vi "ot-spectra-to-flexlogger-test.vi"(1 "Order Settings":T2={"pulses per rev"=1, "trigger level (V)"=2.5, "max order"=64.0, "order resolution"=0.1, "window"=1, "averaging parameters"={"averaging mode"=enum."No averaging", "weighting mode"=enum."Linear", "number of averages"=1, "linear mode"=enum."One shot"}, "order ranges"=[{"start"=0.8, "stop"=1.2}, {"start"=1.8, "stop"=2.2}, {"start"=3.37, "stop"=3.77}, {"start"=3.8, "stop"=4.2}, {"start"=23.8, "stop"=24.2}]}, 4 "Noise (g rms)":dbl=0.01, 5 "Phases (deg)":dbl[](array[numeric])=[30.0, 0.0, 0.0, 0.0, 0.0], 6 "Orders":dbl[](array[numeric])=[1.0, 2.0, 3.57, 4.0, 24.0], 7 "Amplitudes (g pk)":dbl[](array[numeric])=[0.5, 0.2, 0.1, 0.05, 0.3], 8 "error in (no error)":errorcluster, 9 "Duration (s)":dbl=30.0, 10 "Ramps":T3(array[cluster]), 11 "Base RPM":dbl=3000.0) -> (0 "error out":errorcluster, 2 "True RPM":dbl[](array[numeric]), 3 "Tach RPM":dbl[](array[numeric]))   [LabVIEW 2026]
doc: "Unit-test harness for OT Spectra to FlexLogger.vi, fed block by block by the S&V order power spectrum chain of the NI example (Analog Tacho Process, Convert to Even Angle, Order Power Spectrum). Synthesises accel (sum of order sines, peak amplitudes, uniform noise) and a 1 ppr 0-5 V square tach (rising edge at shaft angle 0) for rpm(t) = Base RPM + sum of linear ramps, cuts it into 0.1 s blocks (5120 S @ 51.2 kS/s) and calls OrderPowerSpectrum.vi block by block like FlexLogger Process.vi does (Data In = [accel, tach], reset? TRUE on block 0). Returns NUMERIC arrays only: Values [blocks x (2 + order ranges)] = RPM, order amplitudes (g rms), Spectrum Valid, True RPM at each block centre."
uses:
  <vilib>/addons/Sound and Vibration/Order Analysis/Tach Process/OAT Analog Tacho Process (1 Tacho).vi
  <vilib>/addons/Sound and Vibration/Order Analysis/Resample Order Tracking/OAT Convert to Even Angle Signal (1 Channel).vi
  <vilib>/addons/Sound and Vibration/Order Analysis/Resample Order Tracking/OAT Order Power Spectrum (1 Channel).vi
  <vilib>/addons/Sound and Vibration/Order Analysis/Tach Process/SoundVib_TachProcess.lvlib
  <vilib>/addons/Sound and Vibration/Order Analysis/Resample Order Tracking/SoundVib_OrderTracking.lvlib
panel:
  out "Waveforms per Block":i32[](array[numeric])
  out "Values":dbl[][](array[numeric])
  in  "Settings":T1={"channels"=1, "orders"=[1.0, 2.0, 24.0], "band half-width (orders)"=0.2, "window ENBW (bins)"=1.5}
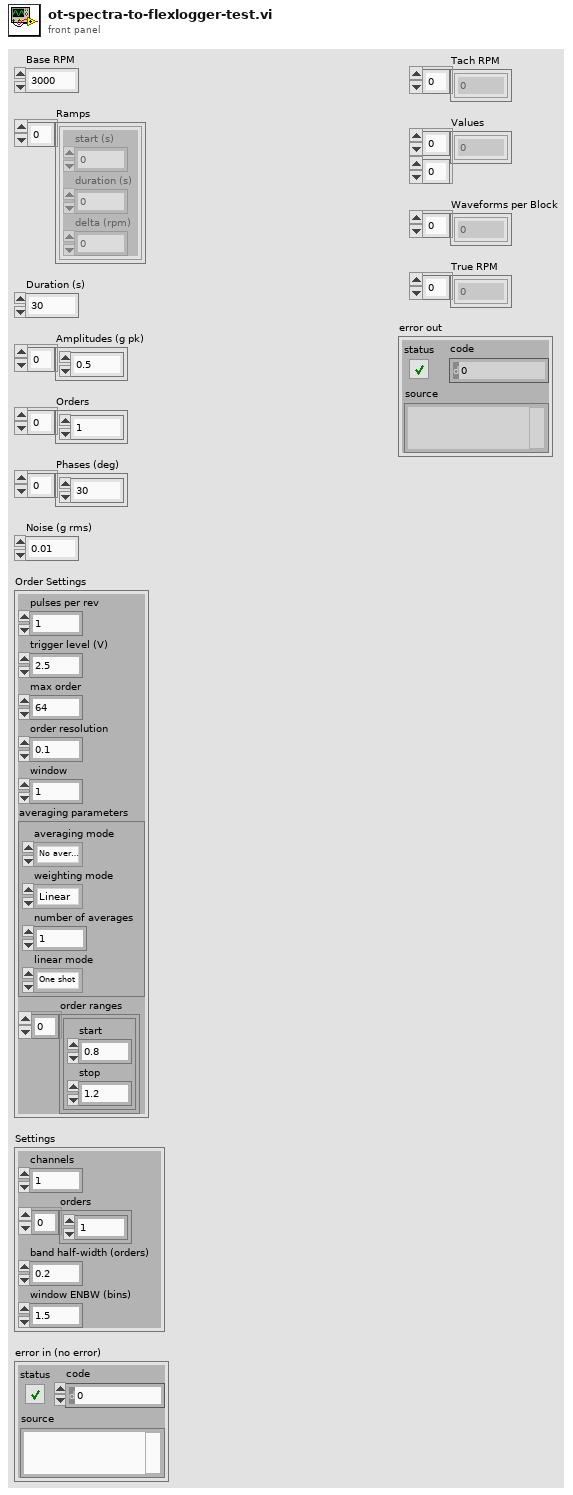
[diagram p1: front panel]
types:
  T1 = cluster{"channels":i32, "orders":dbl[], "band half-width (orders)":dbl, "window ENBW (bins)":dbl}
  T2 = cluster{"pulses per rev":i32, "trigger level (V)":dbl, "max order":dbl, "order resolution":dbl, "window":u32, "averaging parameters":cluster{"averaging mode":enum16{"No averaging", "Vector averaging", "RMS averaging", "Peak hold"}, "weighting mode":enum16{"Linear", "Exponential"}, "number of averages":u32, "linear mode":enum16{"One shot", "Auto restart"}}, "order ranges":cluster{"start":dbl, "stop":dbl}[]}
  T3 = cluster{"start (s)":dbl, "duration (s)":dbl, "delta (rpm)":dbl}[]
  T4 = cluster{"averaging mode":enum16{"No averaging", "Vector averaging", "RMS averaging", "Peak hold"}, "weighting mode":enum16{"Linear", "Exponential"}, "number of averages":u32, "linear mode":enum16{"One shot", "Auto restart"}}
  T5 = typedef "SoundVib_TachProcess.lvlib/speed profile.ctl" = cluster{"time [s]":dbl[], "speed [RPM]":dbl[]}
  T6 = typedef "svc_Resampled Channel Info.ctl" = cluster{"channel name":string, "description":string, " channel info":T7}
  T7 = typedef "svc_Channel Info.ctl" = cluster{"sensor sensitivity":dbl, "engineering units":T8, "dB reference":dbl, "custom label":string, "weighting filter":T9, "pregain":dbl}
  T8 = typedef "svc_Engineering Units Text Ring.ctl" = u16
  T9 = typedef "svc_Weighting Filter Text Ring.ctl" = u16
  T10 = cluster{"order 0":dbl, "delta order":dbl, "magnitude":dbl[]}
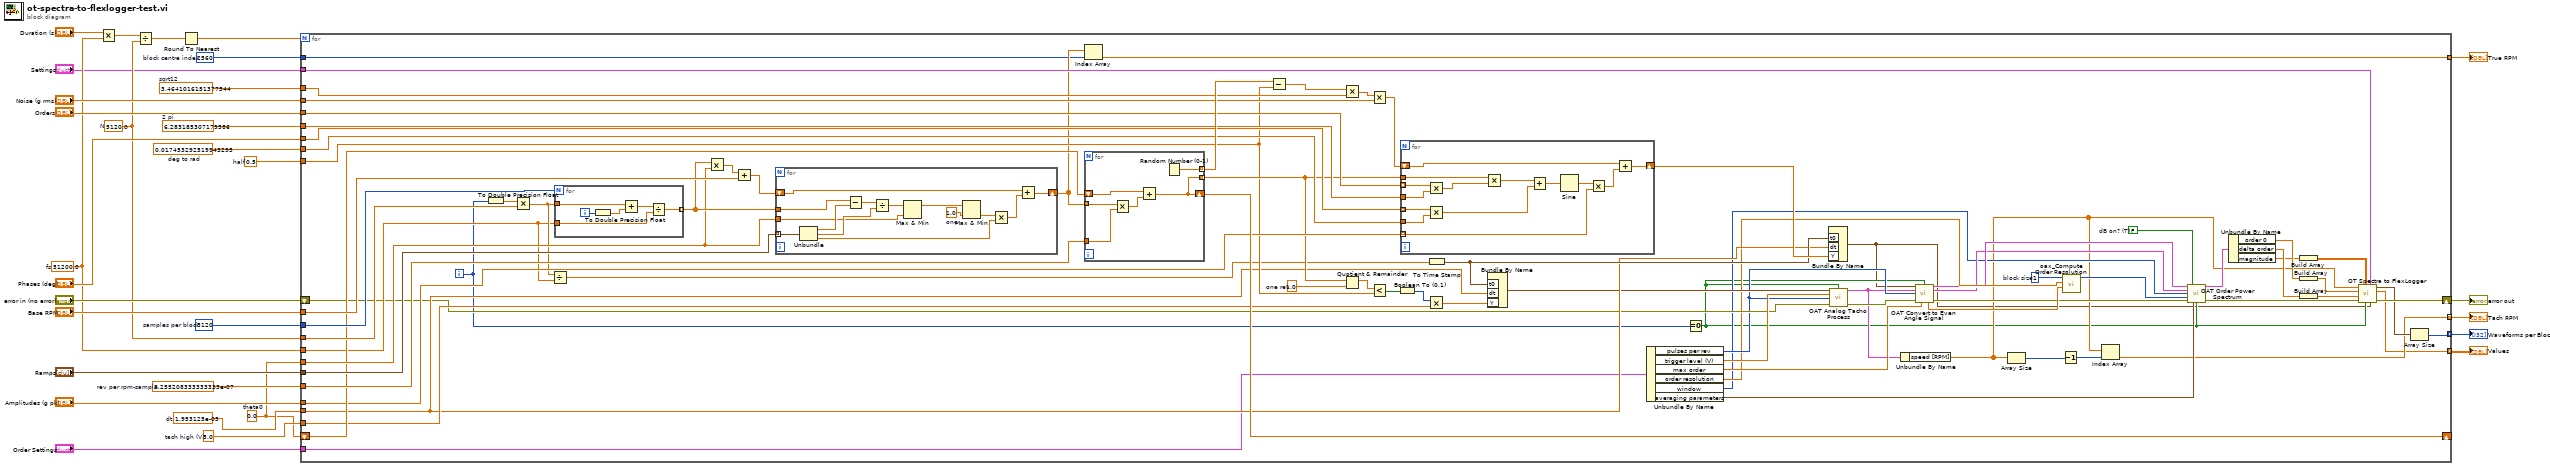
[diagram p0: block diagram]
diagram:
  w9 = 2560  # block centre index
  w10 = 5.0  # tach high (V)
  w11 = 6.283185307179586  # 2 pi
  w12 = 0.017453292519943295  # deg to rad
  w13 = 0.5  # half
  w14 = 3.4641016151377544  # sqrt12
  w15 = 1.953125e-05  # dt
  w16 = 3.255208333333333e-07  # rev per rpm-sample
  w8 = 0.0  # theta0
  w17 = 5120.0  # N
  w18 = 5120  # samples per block
  w19 = 51200.0  # fs
  n1 = Multiply(x="Duration (s)", y=w19) -> (x*y=w29:dbl)
  n2 = Divide(x=w29, y=w17) -> (x/y=w28:dbl)
  n3 = Round To Nearest(number=w28) -> (nearest integer value=w6:dbl)
  n4 = for {
    N: w6 -> [_]
    shift-right: [w98] -> _
    shift-left: w8 -> [w97]
    shift-right: [w39] -> w1
    shift-left: "error in (no error)" -> [w68]
    tunnel: "Base RPM" -> [w104]
    tunnel: "Ramps" -> [w103]
    tunnel: "Amplitudes (g pk)" -> [w90]
    tunnel: "Orders" -> [w91]
    tunnel: "Phases (deg)" -> [w89]
    tunnel: "Noise (g rms)" -> [w92]
    tunnel: "Order Settings" -> [w71]
    tunnel: w19 -> [w77]
    tunnel: w18 -> [w106]
    tunnel: w17 -> [w107]
    tunnel: w16 -> [w99]
    tunnel: w15 -> [w73]
    tunnel: w14 -> [w94]
    tunnel: w13 -> [w82]
    tunnel: w12 -> [w87]
    tunnel: w11 -> [w88]
    tunnel: w10 -> [w79]
    tunnel: w9 -> [w36]
    tunnel: w8 -> [w101]
    tunnel: "Settings" -> [w42]
    tunnel: [w35] -> w5 mode=indexing
    tunnel: [w34] -> w4 mode=indexing
    tunnel: [w33] -> w3 mode=indexing
    tunnel: [w32] -> w2 mode=indexing
    i -> [w31]
    w60 = FALSE  # dB on? (T)
    w64 = 1  # block size
    w84 = 1.0  # one rev
    n5 = To Double Precision Float(number=w31) -> (double precision float=w108:dbl)
    n6 = Multiply(x=w108, y=w107) -> (x*y=w78:dbl)
    n7 = Divide(x=w78, y=w77) -> (x/y=w76:dbl)
    n8 = for {
      N: w106 -> [_]
      tunnel: w78 -> [w148]
      tunnel: w77 -> [w145]
      tunnel: [w144] -> w102 mode=indexing
      i -> [w143]
      n9 = To Double Precision Float(number=w143) -> (double precision float=w147:dbl)
      n10 = Add(x=w148, y=w147) -> (x+y=w146:dbl)
      n11 = Divide(x=w146, y=w145) -> (x/y=w144:dbl)
    }
    n12 = Multiply(x=w102, y=w101) -> (x*y=w105:dbl[])
    n13 = Add(x=w105, y=w104) -> (x+y=w100:dbl[])
    n14 = for {
      tunnel: w103 -> [w142] mode=indexing
      tunnel: w102 -> [w141]
      tunnel: w101 -> [w136]
      shift-right: [w129] -> w37
      shift-left: w100 -> [w131]
      w134 = 1.0  # one
      n15 = Unbundle(w142) -> ("start (s)"=w140:dbl, "duration (s)"=w138:dbl, "delta (rpm)"=w132:dbl)
      n16 = Subtract(x=w141, y=w140) -> (x-y=w139:dbl[])
      n17 = Divide(x=w139, y=w138) -> (x/y=w137:dbl[])
      n18 = Max & Min(x=w137, y=w136) -> (max(x,y)=w135:dbl[])  [unwired: 1 out]
      n19 = Max & Min(x=w135, y=w134) -> (min(x,y)=w133:dbl[])  [unwired: 1 out]
      n20 = Multiply(x=w133, y=w132) -> (x*y=w130:dbl[])
      n21 = Add(x=w131, y=w130) -> (x+y=w129:dbl[])
    }
    n22 = Index Array(array=w37, index=w36) -> (element=w32:dbl)
    n23 = for {
      tunnel: w37 -> [w128] mode=indexing
      tunnel: w99 -> [w127]
      shift-right: [w124] -> w98
      shift-left: w97 -> [w126]
      tunnel: [w124] -> w85 mode=indexing
      tunnel: [w123] -> w96 mode=indexing
      n24 = Multiply(x=w128, y=w127) -> (x*y=w125:dbl)
      n25 = Add(x=w126, y=w125) -> (x+y=w124:dbl)
      n26 = Random Number (0-1)() -> (number: 0 to 1=w123:dbl)
    }
    n27 = Subtract(x=w96, y=w82) -> (x-y=w95:dbl[])
    n28 = Multiply(x=w95, y=w94) -> (x*y=w93:dbl[])
    n29 = Quotient & Remainder(x=w85, y=w84) -> (x-y*floor(x/y)=w83:dbl[])  [unwired: 1 out]
    n30 = Multiply(x=w93, y=w92) -> (x*y=w86:dbl[])
    n31 = Less?(x=w83, y=w82) -> (x < y?=w81:bool[])
    n32 = Boolean To (0,1)(Boolean=w81) -> (0, 1=w80:i16[])
    n33 = for {
      tunnel: w91 -> [w122] mode=indexing
      tunnel: w90 -> [w112] mode=indexing
      tunnel: w89 -> [w118] mode=indexing
      tunnel: w85 -> [w120]
      tunnel: w88 -> [w121]
      tunnel: w87 -> [w117]
      shift-right: [w109] -> w75
      shift-left: w86 -> [w111]
      n34 = Multiply(x=w122, y=w121) -> (x*y=w119:dbl)
      n35 = Multiply(x=w118, y=w117) -> (x*y=w115:dbl)
      n36 = Multiply(x=w120, y=w119) -> (x*y=w116:dbl[])
      n37 = Add(x=w116, y=w115) -> (x+y=w114:dbl[])
      n38 = Sine(x=w114) -> (sin(x)=w113:dbl[])
      n39 = Multiply(x=w113, y=w112) -> (x*y=w110:dbl[])
      n40 = Add(x=w111, y=w110) -> (x+y=w109:dbl[])
    }
    n41 = Multiply(x=w80, y=w79) -> (x*y=w72:dbl[])
    n42 = To Time Stamp(1:w76) -> (0:w74:timestamp)
    n43 = Bundle By Name("t0"=w74, "dt"=w73, "Y"=w72) -> (w70:waveform(dbl))  [unwired: 1 in]
    n44 = Unbundle By Name(w71) -> ("pulses per rev"=w67:i32, "trigger level (V)"=w69:dbl, "max order"=w66:dbl, "order resolution"=w63:dbl, "window"=w58:u32, "averaging parameters"=w55:T4)
    n45 = Equal To 0?(x=w31) -> (x = 0?=w43:bool)
    n46 = Bundle By Name("t0"=w74, "dt"=w73, "Y"=w75) -> (w41:waveform(dbl))  [unwired: 1 in]
    n47 = call-poly <vilib>:"OAT Analog Tacho Process.vi"("analog tacho signal"=w70, "reset? (F)"=w43, "threshold (auto)"=w69, "pulse/revolution (1)"=w67, "error in (no error)"=w68) -> ("speed profile"=w54:T5, "error out"=w65:errorcluster)  [unwired: 6 in, 3 out]
    n48 = Unbundle By Name(w54) -> ("speed [RPM]"=w47:dbl[])
    n49 = call-poly <vilib>:"OAT Convert to Even Angle Signal.vi"("scaled signal [EU]"=w41, "reset? (F)"=w43, "speed profile"=w54, "pulse/revolution (1)"=w67, "error in (no error)"=w65, "max order (auto)"=w66) -> ("even-angle signal"=w61:cluster{"r0":dbl, "dr":dbl, "Y":dbl[]}, "even-angle channel info"=w59:T6, "actual max order"=w62:dbl, "error out"=w56:errorcluster)  [unwired: 5 in, 1 out]
    n50 = Array Size(array=w47) -> (size(s)=w53:i32)
    n51 = Decrement(x=w53) -> (x-1=w52:i32)
    n52 = call <vilib>:"oax_Compute Order Resolution.vi"("actual max order"=w62, "order resolution"=w63, "block size"=w64) -> ("block size out"=w57:i32)  [unwired: 7 in, 1 out]
    n53 = Index Array(array=w47, index=w52) -> (element=w35:dbl)
    n54 = call-poly <vilib>:"OAT Order Power Spectrum.vi"("even-angle signal"=w61, "dB on? (T)"=w60, "even-angle channel info"=w59, "window"=w58, "block size"=w57, "error in (no error)"=w56, "averaging parameters"=w55, "restart averaging? (F)"=w43) -> ("order power spectrum"=w51:T10, "error out"=w40:errorcluster)  [unwired: 1 in, 5 out]
    n55 = Unbundle By Name(w51) -> ("order 0"=w50:dbl, "delta order"=w49:dbl, "magnitude"=w48:dbl[])
    n56 = Build Array(w48) -> (w44:dbl[][])
    n57 = Build Array(w50) -> (w46:dbl[])
    n58 = Build Array(w49) -> (w45:dbl[])
    n59 = call "OT Spectra to FlexLogger.vi"("Timing Reference"=w41, "Settings"=w42, "reset? (F)"=w43, "magnitude"=w44, "error in (no error)"=w40, "delta order"=w45, "order 0"=w46, "speed [RPM]"=w47) -> ("error out"=w39:errorcluster, "Values"=w34:dbl[], "Array of Waveforms"=w38:waveform(dbl)[])  [unwired: 1 in]
    n60 = Array Size(array=w38) -> (size(s)=w33:i32)
  }
  "Tach RPM" <- w5
  "Values" <- w4
  "Waveforms per Block" <- w3
  "True RPM" <- w2
  "error out" <- w1
